vi "am filter.vi"() -> ()   [LabVIEW 2021]
uses:
  <vilib>/express/express analysis/Spectral/Block/exnSpectralBlock spectral measurements RMS poly.vi
  <vilib>/express/express analysis/Spectral/Block/exnSpectralBlock spectral measurements RMS DDT.vi
  <vilib>/express/express analysis/Spectral/XNode/ExpressSpectralMeasurementsBlockNode.xnode
panel:
  out "Waveform Graph 5":dynamicdata(graph)
  out "Waveform Graph 4":dynamicdata(graph)
  out "Waveform Graph 3":dynamicdata(graph)
  in  "am":dbl=15.0 caption="Amplitude"
  in  "ac":dbl=15.0 caption="Amplitude"
  out "Waveform Graph 2":dynamicdata(graph)
  out "Waveform Graph":dynamicdata(graph)
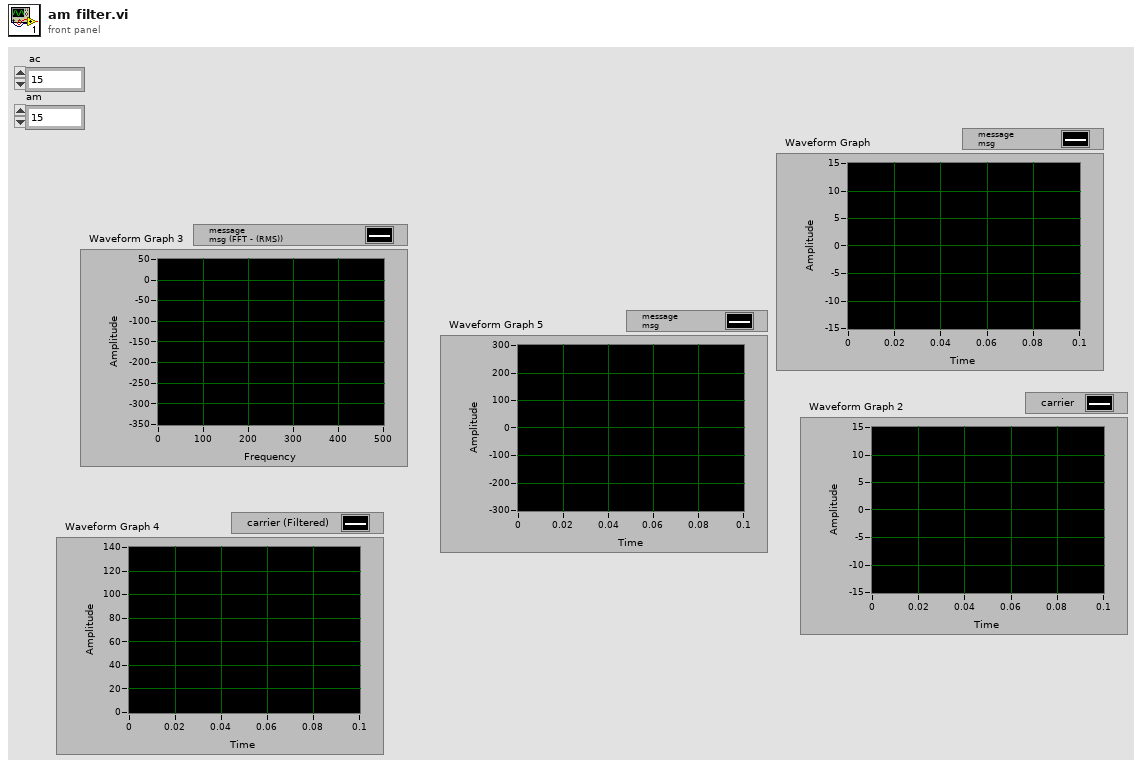
[diagram p1: front panel]
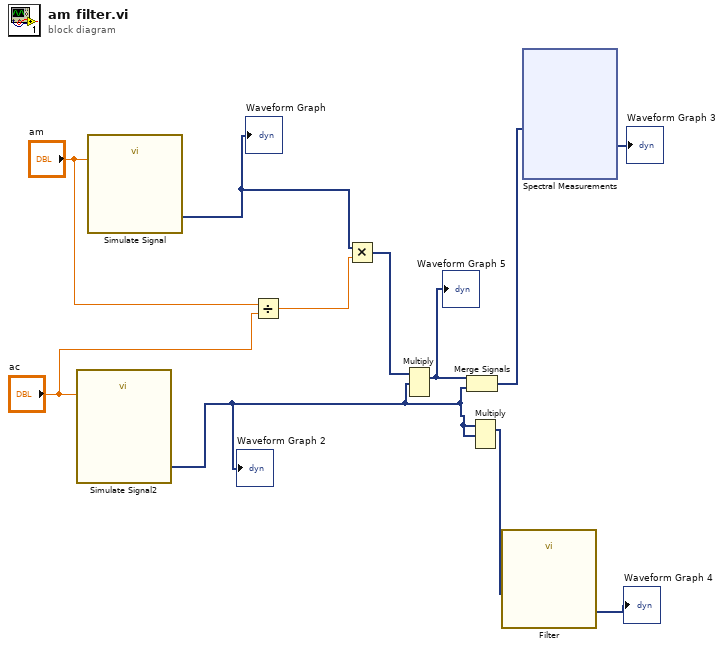
[diagram p0: block diagram]
diagram:
  n1 = call "Simulate Signal2"("Amplitude"="ac") -> ("carrier"=w1:dynamicdata)  [unwired: 13 in, 1 out]
  "Waveform Graph 2" <- w1
  n2 = call "Simulate Signal"("Amplitude"="am") -> ("message\nmsg"=w9:dynamicdata)  [unwired: 13 in, 1 out]
  "Waveform Graph" <- w9
  n3 = Divide(x="am", y="ac") -> (x/y=w8:dbl)
  n4 = Multiply(x=w9, y=w8) -> (x*y=w7:dynamicdata)
  n5 = Multiply(1:w1, 2:w7) -> (0:w3:dynamicdata)  [unwired: 1 in, 1 out]
  "Waveform Graph 5" <- w3
  n6 = Merge Signals(w3, w1) -> (w2:dynamicdata)
  n7 = Multiply(1:w1, 2:w1) -> (0:w6:dynamicdata)  [unwired: 1 in, 1 out]
  n8 = call "Filter"("Signal"=w6) -> ("Filtered Signal"=→"Waveform Graph 4":dynamicdata)  [unwired: 9 in, 1 out]
  n9 = xnode "Spectral Measurements"("Signals"=w2) -> ("FFT - (RMS)"=→"Waveform Graph 3":dynamicdata)  [unwired: 1 in, 2 out]
